vi "Check If Discovery Service is Running.vi"(8 "error in":errorcluster) -> (0 "error out":errorcluster, 3 "discovery service running?":bool)   [LabVIEW 2021, in "MeasurementServerTests.lvlib"]
uses:
  MeasurementServerTests.lvlib
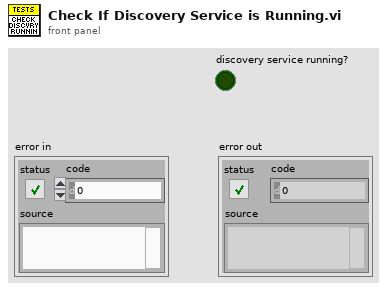
[diagram p1: front panel]
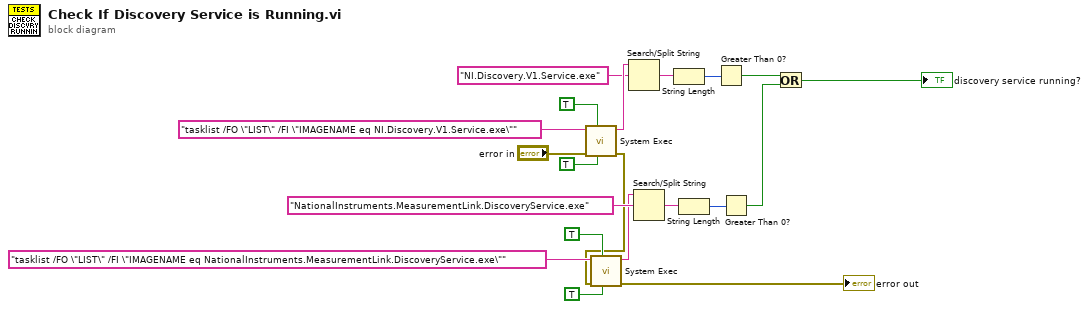
[diagram p0: block diagram]
diagram:
  n1 = call <vilib>:"System Exec.vi"("run minimized? (F)"=TRUE, "wait until completion? (T)"=TRUE, "error in (no error)"="error in", "command line"="tasklist /FO \"LIST\" /FI \"IMAGENAME eq NI.Discovery.V1.Service.exe\"") -> ("error out"=w2:errorcluster, "standard output"=w16:string)  [unwired: 4 in, 2 out]
  n2 = call <vilib>:"System Exec.vi"("run minimized? (F)"=TRUE, "wait until completion? (T)"=TRUE, "error in (no error)"=w2, "command line"="tasklist /FO \"LIST\" /FI \"IMAGENAME eq NationalInstruments.MeasurementLink.DiscoveryService.exe\"") -> ("error out"=→"error out":errorcluster, "standard output"=w9:string)  [unwired: 4 in, 2 out]
  n3 = Search/Split String(string=w16, search string/char (-)="NI.Discovery.V1.Service.exe") -> (match + rest of string=w14:string)  [unwired: 1 in, 2 out]
  n4 = Search/Split String(string=w9, search string/char (-)="NationalInstruments.MeasurementLink.DiscoveryService.exe") -> (match + rest of string=w11:string)  [unwired: 1 in, 2 out]
  n5 = String Length(string=w14) -> (length=w13:i32)
  n6 = String Length(string=w11) -> (length=w12:i32)
  n7 = Greater Than 0?(x=w13) -> (x > 0?=w5:bool)
  n8 = Greater Than 0?(x=w12) -> (x > 0?=w3:bool)
  n9 = Or(x=w5, y=w3) -> (x .or. y?=→"discovery service running?":bool)
